vi "Read Parameter.vi"(8 "error in (no error)":errorcluster, 11 "PGJDPMapper in":refnum<class "Mapper.lvclass">) -> (0 "error out":errorcluster, 2 "DynamicParameters out":refnum<class "DynamicParameters.lvclass">, 3 "PGJDPMapper out":refnum<class "Mapper.lvclass">)   [LabVIEW 2020, in "ORM_pgsql_jdp.lvlib" / "Mapper.lvclass"]
uses:
  Mapper.lvclass
  <vilib>/Viviota/shared/ORM.lvlibp/DynamicParameters/DynamicParameters.lvclass
  PGJDPParameter/Parameter.lvclass
  C:/Program Files/National Instruments/LabVIEW 2020/vi.lib/Viviota/shared/ORM.lvlibp/DynamicParameters/DynamicParameters.lvclass
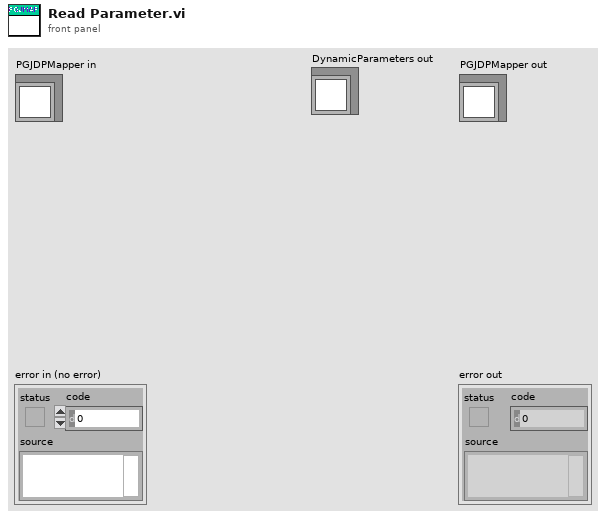
[diagram p1: front panel]
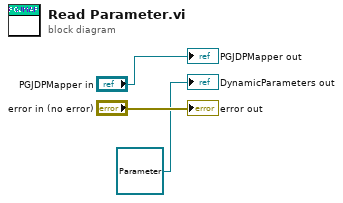
[diagram p0: block diagram]
diagram:
  "error out" <- "error in (no error)"
  "PGJDPMapper out" <- "PGJDPMapper in"
  "DynamicParameters out" <- refnum<class "Parameter.lvclass"> refnum ("ORM_pgsql_jdp.lvlib:PGJDPParameter.lvclass")
